vi "test_FindProjects.vi"() -> (3 "Pass?":bool)   [LabVIEW 2019, in "Tests.SolutionBuilder.lvlib"]
uses:
  Tests.SolutionBuilder.lvlib
  SolutionBuilder/SolutionBuilder.lvclass
  SolutionBuilder/ProjectItem/ProjectItem.lvclass
panel:
  out "test results":u32 format="%010b"
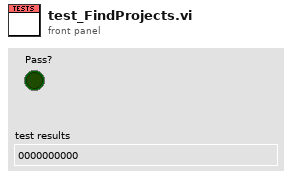
[diagram p1: front panel]
types:
  T1 = typedef "SolutionBuilder.lvlib/SolutionBuilder.lvclass/ProjectItemMap.ctl" = map{path, refnum<class "ProjectItem.lvclass">[]}
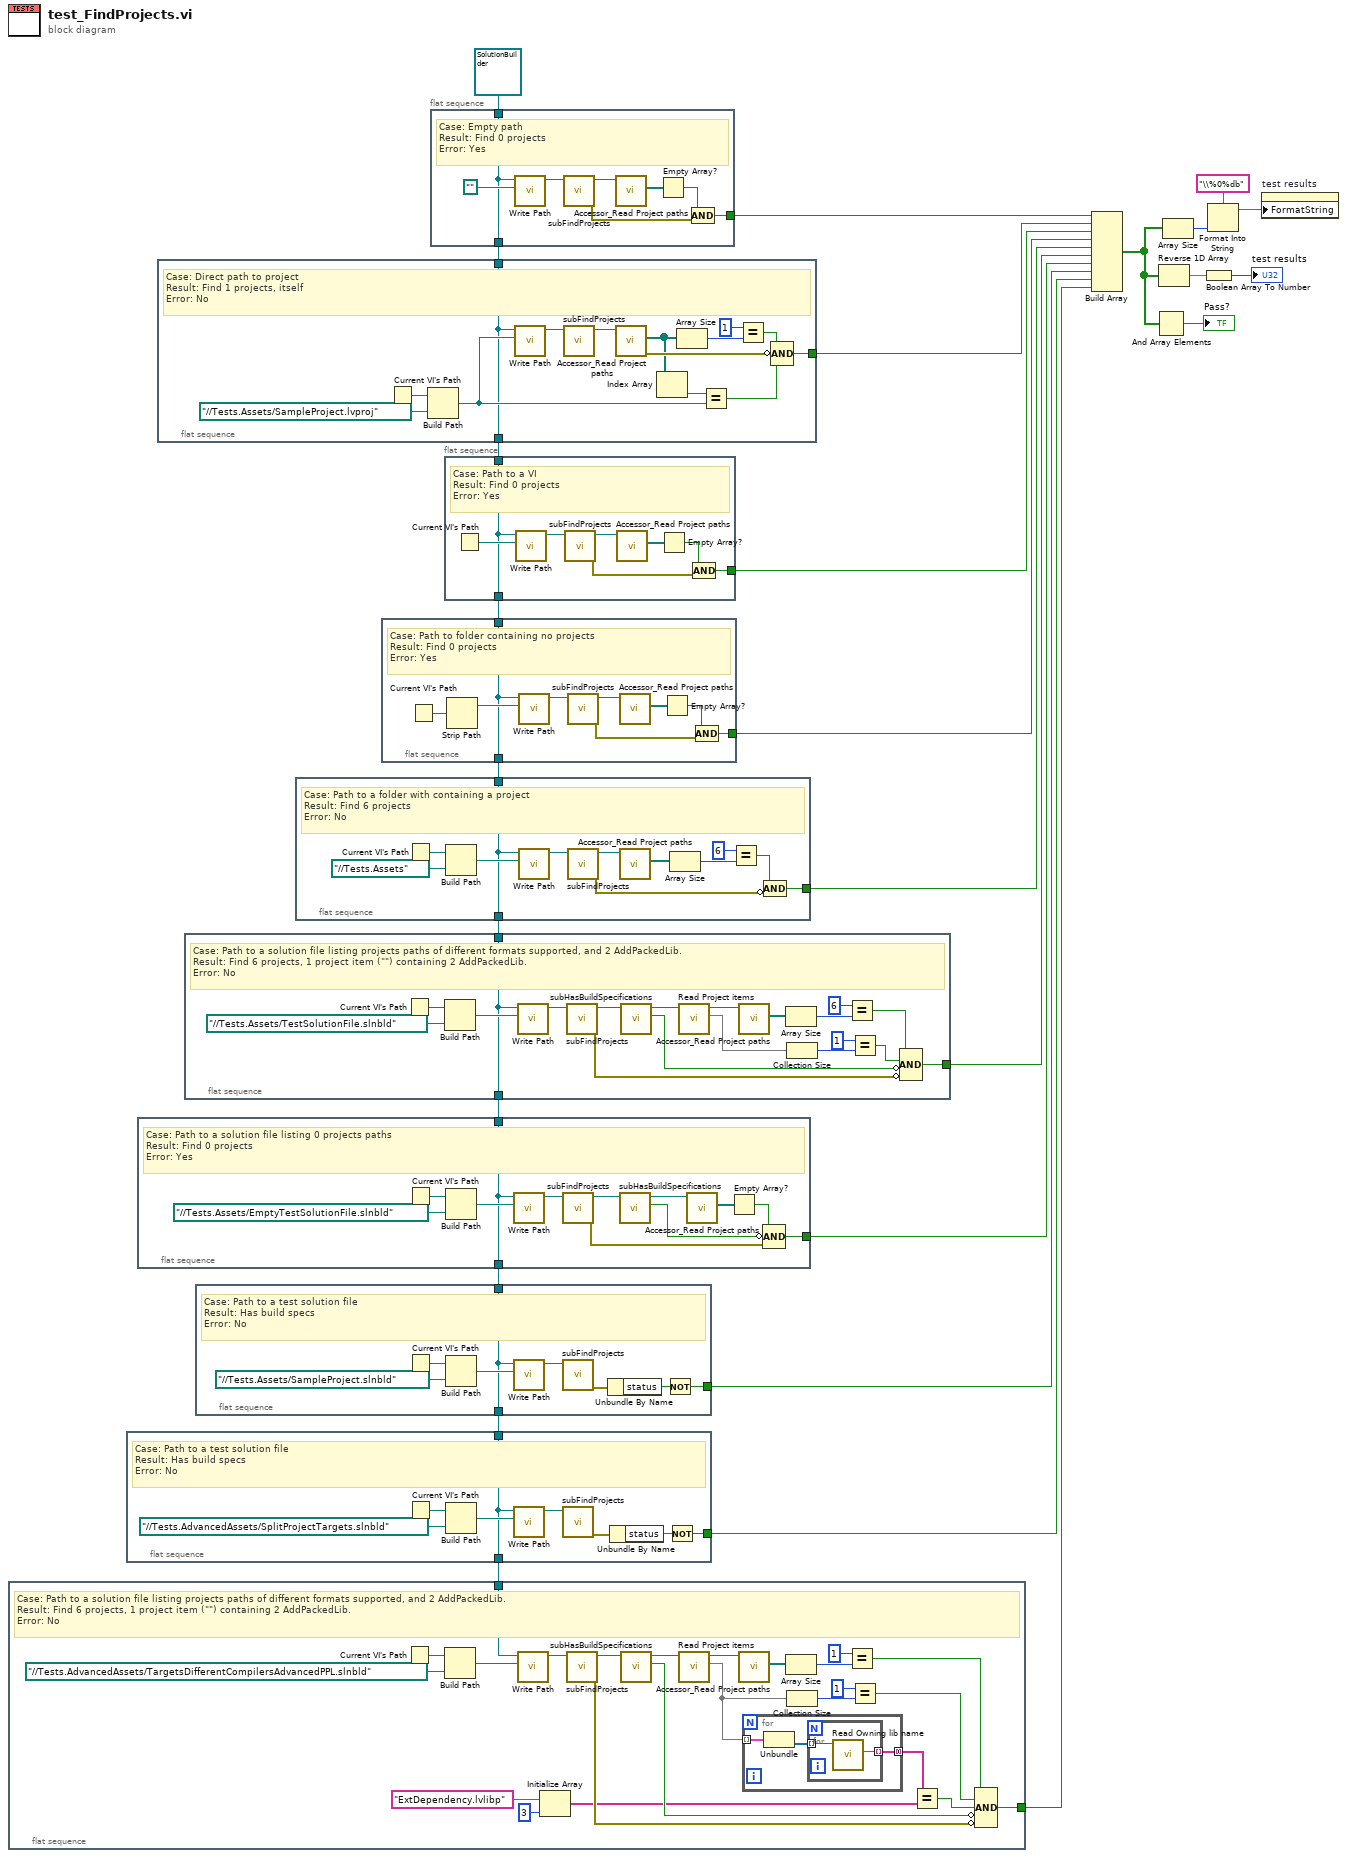
[diagram p0: block diagram]
diagram:
  n1 = flat-sequence {
    tunnel: [w45] -> w1
    tunnel: w2 -> [w41]
    frame #0 {
      # "Case: Path to a solution file listing projects paths of different formats supported, and 2 AddPackedLib. \nResult: Find 6 projects, 1 project item (\"\") containing 2 AddPackedLib.\nError: No"
      n2 = Current VI's Path() -> (path=w50:path)
      n3 = Build Path(base path=w50, name or relative path=path "../../Tests.AdvancedAssets/TargetsDifferentCompilersAdvancedPPL.slnbld" ("Path")) -> (appended path=w42:path)
      n4 = call "Write Path.vi"("Path"=w42, "SolutionBuilder in"=w41) -> ("SolutionBuilder out"=w51:refnum<class "SolutionBuilder.lvclass">)  [unwired: 9 in]
      n5 = Initialize Array("ExtDependency.lvlibp" ("Owning lib name"), 3 ("dimension size")) -> (w30:string[])
      n6 = call "subFindProjects.vi"("SolutionBuilder in"=w51) -> ("error out"=w44:errorcluster, "SolutionBuilder out"=w36:refnum<class "SolutionBuilder.lvclass">)  [unwired: 9 in]
      n7 = call "subHasBuildSpecifications.vi"("SolutionBuilder in"=w36) -> ("Has specs?"=w34:bool, "SolutionBuilder out"=w35:refnum<class "SolutionBuilder.lvclass">)  [unwired: 8 in, 1 out]
      n8 = call "Read Project items.vi"("SolutionBuilder in"=w35) -> ("Project items"=w33:T1, "SolutionBuilder out"=w40:refnum<class "SolutionBuilder.lvclass">)  [unwired: 9 in]
      n9 = call "Accessor_Read Project paths.vi"("SolutionBuilder in"=w40) -> ("Project paths"=w43:path[])  [unwired: 8 in, 2 out]
      n10 = for {
        tunnel: w33 -> [w54] mode=indexing
        tunnel: [w52] -> w29 mode=concatenating
        n11 = Unbundle(w54) -> ("ProjectItems"=w53:refnum<class "ProjectItem.lvclass">[])  [unwired: 1 out]
        n12 = for {
          tunnel: w53 -> [w56] mode=indexing
          tunnel: [w55] -> w52 mode=indexing
          n13 = call "Read Owning lib name.vi"("ProjectItem in"=w56) -> ("Owning lib name"=w55:string)  [unwired: 9 in, 1 out]
        }
      }
      n14 = Array Size(array=w43) -> (size(s)=w48:i32)
      n15 = Collection Size(1:w33) -> (0:w38:i32)
      n16 = Equal?(x=1, y=w48) -> (x = y?=w46:bool)
      n17 = Equal?(x=1, y=w38) -> (x = y?=w37:bool)
      n18 = Equal?(x=w29, y=w30) -> (x = y?=w28:bool)
      n19 = Compound Arithmetic op=AND(w46, w37, w28, invert w34, invert w44) -> (w45:bool)
    }
  }
  n20 = flat-sequence {
    tunnel: [w58] -> w3
    tunnel: w5 -> [w57]
    tunnel: [w57] -> w2
    frame #0 {
      # "Case: Path to a test solution file \nResult: Has build specs\nError: No"
      n21 = Current VI's Path() -> (path=w62:path)
      n22 = Build Path(base path=w62, name or relative path=path "../../Tests.AdvancedAssets/SplitProjectTargets.slnbld" ("Path")) -> (appended path=w61:path)
      n23 = call "Write Path.vi"("Path"=w61, "SolutionBuilder in"=w57) -> ("SolutionBuilder out"=w64:refnum<class "SolutionBuilder.lvclass">)  [unwired: 9 in]
      n24 = call "subFindProjects.vi"("SolutionBuilder in"=w64) -> ("error out"=w59:errorcluster)  [unwired: 9 in, 1 out]
      n25 = Unbundle By Name(w59) -> ("status"=w60:bool)
      n26 = Not(x=w60) -> (.not. x?=w58:bool)
    }
  }
  n27 = flat-sequence {
    tunnel: [w69] -> w14
    tunnel: w8 -> [w65]
    tunnel: [w65] -> w6
    frame #0 {
      # "Case: Path to a solution file listing 0 projects paths\nResult: Find 0 projects\nError: Yes"
      n28 = Current VI's Path() -> (path=w71:path)
      n29 = Build Path(base path=w71, name or relative path=path "../../Tests.Assets/EmptyTestSolutionFile.slnbld" ("Path")) -> (appended path=w70:path)
      n30 = call "Write Path.vi"("Path"=w70, "SolutionBuilder in"=w65) -> ("SolutionBuilder out"=w73:refnum<class "SolutionBuilder.lvclass">)  [unwired: 9 in]
      n31 = call "subFindProjects.vi"("SolutionBuilder in"=w73) -> ("error out"=w74:errorcluster, "SolutionBuilder out"=w68:refnum<class "SolutionBuilder.lvclass">)  [unwired: 9 in]
      n32 = call "subHasBuildSpecifications.vi"("SolutionBuilder in"=w68) -> ("Has specs?"=w66:bool, "SolutionBuilder out"=w67:refnum<class "SolutionBuilder.lvclass">)  [unwired: 8 in, 1 out]
      n33 = call "Accessor_Read Project paths.vi"("SolutionBuilder in"=w67) -> ("Project paths"=w75:path[])  [unwired: 8 in, 2 out]
      n34 = Empty Array?(array=w75) -> (empty?=w76:bool)
      n35 = Compound Arithmetic op=AND(w76, invert w66, w74) -> (w69:bool)
    }
  }
  n36 = flat-sequence {
    tunnel: [w82] -> w20
    tunnel: w13 -> [w77]
    tunnel: [w77] -> w12
    frame #0 {
      # "Case: Direct path to project\nResult: Find 1 projects, itself\nError: No"
      n37 = Current VI's Path() -> (path=w88:path)
      n38 = Build Path(base path=w88, name or relative path=path "../../Tests.Assets/SampleProject.lvproj" ("Path")) -> (appended path=w79:path)
      n39 = call "Write Path.vi"("Path"=w79, "SolutionBuilder in"=w77) -> ("SolutionBuilder out"=w90:refnum<class "SolutionBuilder.lvclass">)  [unwired: 9 in]
      n40 = call "subFindProjects.vi"("SolutionBuilder in"=w90) -> ("SolutionBuilder out"=w89:refnum<class "SolutionBuilder.lvclass">)  [unwired: 9 in, 1 out]
      n41 = call "Accessor_Read Project paths.vi"("SolutionBuilder in"=w89) -> ("error out"=w83:errorcluster, "Project paths"=w81:path[])  [unwired: 8 in, 1 out]
      n42 = Index Array(array=w81) -> (element=w80:path)  [unwired: 1 in]
      n43 = Array Size(array=w81) -> (size(s)=w86:i32)
      n44 = Equal?(x=w80, y=w79) -> (x = y?=w78:bool)
      n45 = Equal?(x=1, y=w86) -> (x = y?=w84:bool)
      n46 = Compound Arithmetic op=AND(w84, invert w83, w78) -> (w82:bool)
    }
  }
  n47 = flat-sequence {
    tunnel: [w103] -> w16
    tunnel: w9 -> [w99]
    tunnel: [w99] -> w8
    frame #0 {
      # "Case: Path to a solution file listing projects paths of different formats supported, and 2 AddPackedLib. \nResult: Find 6 projects, 1 project item (\"\") containing 2 AddPackedLib.\nError: No"
      n48 = Current VI's Path() -> (path=w108:path)
      n49 = Build Path(base path=w108, name or relative path=path "../../Tests.Assets/TestSolutionFile.slnbld" ("Path")) -> (appended path=w100:path)
      n50 = call "Write Path.vi"("Path"=w100, "SolutionBuilder in"=w99) -> ("SolutionBuilder out"=w109:refnum<class "SolutionBuilder.lvclass">)  [unwired: 9 in]
      n51 = call "subFindProjects.vi"("SolutionBuilder in"=w109) -> ("error out"=w102:errorcluster, "SolutionBuilder out"=w93:refnum<class "SolutionBuilder.lvclass">)  [unwired: 9 in]
      n52 = call "subHasBuildSpecifications.vi"("SolutionBuilder in"=w93) -> ("Has specs?"=w91:bool, "SolutionBuilder out"=w92:refnum<class "SolutionBuilder.lvclass">)  [unwired: 8 in, 1 out]
      n53 = call "Read Project items.vi"("SolutionBuilder in"=w92) -> ("Project items"=w95:T1, "SolutionBuilder out"=w98:refnum<class "SolutionBuilder.lvclass">)  [unwired: 9 in]
      n54 = call "Accessor_Read Project paths.vi"("SolutionBuilder in"=w98) -> ("Project paths"=w101:path[])  [unwired: 8 in, 2 out]
      n55 = Array Size(array=w101) -> (size(s)=w106:i32)
      n56 = Collection Size(1:w95) -> (0:w96:i32)
      n57 = Equal?(x=6, y=w106) -> (x = y?=w104:bool)
      n58 = Equal?(x=1, y=w96) -> (x = y?=w94:bool)
      n59 = Compound Arithmetic op=AND(w104, w94, invert w91, invert w102) -> (w103:bool)
    }
  }
  n60 = flat-sequence {
    tunnel: [w110] -> w4
    tunnel: w6 -> [w113]
    tunnel: [w113] -> w5
    frame #0 {
      # "Case: Path to a test solution file \nResult: Has build specs\nError: No"
      n61 = Current VI's Path() -> (path=w115:path)
      n62 = Build Path(base path=w115, name or relative path=path "../../Tests.Assets/SampleProject.slnbld" ("Path")) -> (appended path=w114:path)
      n63 = call "Write Path.vi"("Path"=w114, "SolutionBuilder in"=w113) -> ("SolutionBuilder out"=w117:refnum<class "SolutionBuilder.lvclass">)  [unwired: 9 in]
      n64 = call "subFindProjects.vi"("SolutionBuilder in"=w117) -> ("error out"=w112:errorcluster)  [unwired: 9 in, 1 out]
      n65 = Unbundle By Name(w112) -> ("status"=w111:bool)
      n66 = Not(x=w111) -> (.not. x?=w110:bool)
    }
  }
  n67 = flat-sequence {
    tunnel: [w120] -> w17
    tunnel: w10 -> [w118]
    tunnel: [w118] -> w9
    frame #0 {
      # "Case: Path to a folder with containing a project\nResult: Find 6 projects\nError: No"
      n68 = Current VI's Path() -> (path=w123:path)
      n69 = Build Path(base path=w123, name or relative path=path "../../Tests.Assets" ("Path")) -> (appended path=w129:path)
      n70 = call "Write Path.vi"("Path"=w129, "SolutionBuilder in"=w118) -> ("SolutionBuilder out"=w121:refnum<class "SolutionBuilder.lvclass">)  [unwired: 9 in]
      n71 = call "subFindProjects.vi"("SolutionBuilder in"=w121) -> ("error out"=w119:errorcluster, "SolutionBuilder out"=w122:refnum<class "SolutionBuilder.lvclass">)  [unwired: 9 in]
      n72 = call "Accessor_Read Project paths.vi"("SolutionBuilder in"=w122) -> ("Project paths"=w128:path[])  [unwired: 8 in, 2 out]
      n73 = Array Size(array=w128) -> (size(s)=w125:i32)
      n74 = Equal?(x=6, y=w125) -> (x = y?=w127:bool)
      n75 = Compound Arithmetic op=AND(w127, invert w119) -> (w120:bool)
    }
  }
  n76 = flat-sequence {
    tunnel: [w131] -> w18
    tunnel: w11 -> [w130]
    tunnel: [w130] -> w10
    frame #0 {
      # "Case: Path to folder containing no projects\nResult: Find 0 projects\nError: Yes"
      n77 = Current VI's Path() -> (path=w133:path)
      n78 = Strip Path(path=w133) -> (stripped path=w132:path)  [unwired: 1 out]
      n79 = call "Write Path.vi"("Path"=w132, "SolutionBuilder in"=w130) -> ("SolutionBuilder out"=w138:refnum<class "SolutionBuilder.lvclass">)  [unwired: 9 in]
      n80 = call "subFindProjects.vi"("SolutionBuilder in"=w138) -> ("error out"=w136:errorcluster, "SolutionBuilder out"=w137:refnum<class "SolutionBuilder.lvclass">)  [unwired: 9 in]
      n81 = call "Accessor_Read Project paths.vi"("SolutionBuilder in"=w137) -> ("Project paths"=w135:path[])  [unwired: 8 in, 2 out]
      n82 = Empty Array?(array=w135) -> (empty?=w134:bool)
      n83 = Compound Arithmetic op=AND(w134, w136) -> (w131:bool)
    }
  }
  n84 = flat-sequence {
    tunnel: [w141] -> w21
    tunnel: refnum<class "SolutionBuilder.lvclass"> refnum ("SolutionBuilder in") -> [w139]
    tunnel: [w139] -> w13
    frame #0 {
      # "Case: Empty path\nResult: Find 0 projects\nError: Yes"
      n85 = call "Write Path.vi"("Path"=path "", "SolutionBuilder in"=w139) -> ("SolutionBuilder out"=w146:refnum<class "SolutionBuilder.lvclass">)  [unwired: 9 in]
      n86 = call "subFindProjects.vi"("SolutionBuilder in"=w146) -> ("error out"=w144:errorcluster, "SolutionBuilder out"=w145:refnum<class "SolutionBuilder.lvclass">)  [unwired: 9 in]
      n87 = call "Accessor_Read Project paths.vi"("SolutionBuilder in"=w145) -> ("Project paths"=w143:path[])  [unwired: 8 in, 2 out]
      n88 = Empty Array?(array=w143) -> (empty?=w142:bool)
      n89 = Compound Arithmetic op=AND(w142, w144) -> (w141:bool)
    }
  }
  n90 = flat-sequence {
    tunnel: [w148] -> w19
    tunnel: w12 -> [w147]
    tunnel: [w147] -> w11
    frame #0 {
      # "Case: Path to a VI\nResult: Find 0 projects\nError: Yes"
      n91 = Current VI's Path() -> (path=w149:path)
      n92 = call "Write Path.vi"("Path"=w149, "SolutionBuilder in"=w147) -> ("SolutionBuilder out"=w150:refnum<class "SolutionBuilder.lvclass">)  [unwired: 9 in]
      n93 = call "subFindProjects.vi"("SolutionBuilder in"=w150) -> ("error out"=w152:errorcluster, "SolutionBuilder out"=w151:refnum<class "SolutionBuilder.lvclass">)  [unwired: 9 in]
      n94 = call "Accessor_Read Project paths.vi"("SolutionBuilder in"=w151) -> ("Project paths"=w153:path[])  [unwired: 8 in, 2 out]
      n95 = Empty Array?(array=w153) -> (empty?=w154:bool)
      n96 = Compound Arithmetic op=AND(w154, w152) -> (w148:bool)
    }
  }
  n97 = Build Array(w21, w20, w19, w18, w17, w16, w14, w4, w3, w1) -> (w25:bool[])
  n98 = And Array Elements(Boolean array=w25) -> (logical AND=→"Pass?":bool)
  n99 = Reverse 1D Array(array=w25) -> (reversed array=w7:bool[])
  n100 = Array Size(array=w25) -> (size(s)=w23:i32)
  n101 = Boolean Array To Number(Boolean array=w7) -> (number=→"test results":u32)
  n102 = Format Into String(format string="\\%0%db", w23) -> (resulting string=w22:string)  [unwired: 2 in, 1 out]
  n103 = property on="test results" class="DigNum (strict)"("FormatString"=w22) -> ()  [unwired: 2 in, 2 out]
